vi "BUILD_install and upload core.vi"(6 "Buildlog":path, 8 "error in":errorcluster, 9 "args":string[](array[string]), 11 "vip built path":path) -> (0 "error out":errorcluster)   [LabVIEW 2010]
uses:
  <vilib>/JKI/VIPM API/VIPM API_vipm_api.lvlib
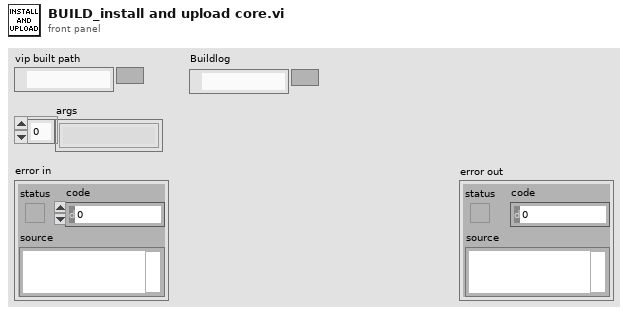
[diagram p1: front panel]
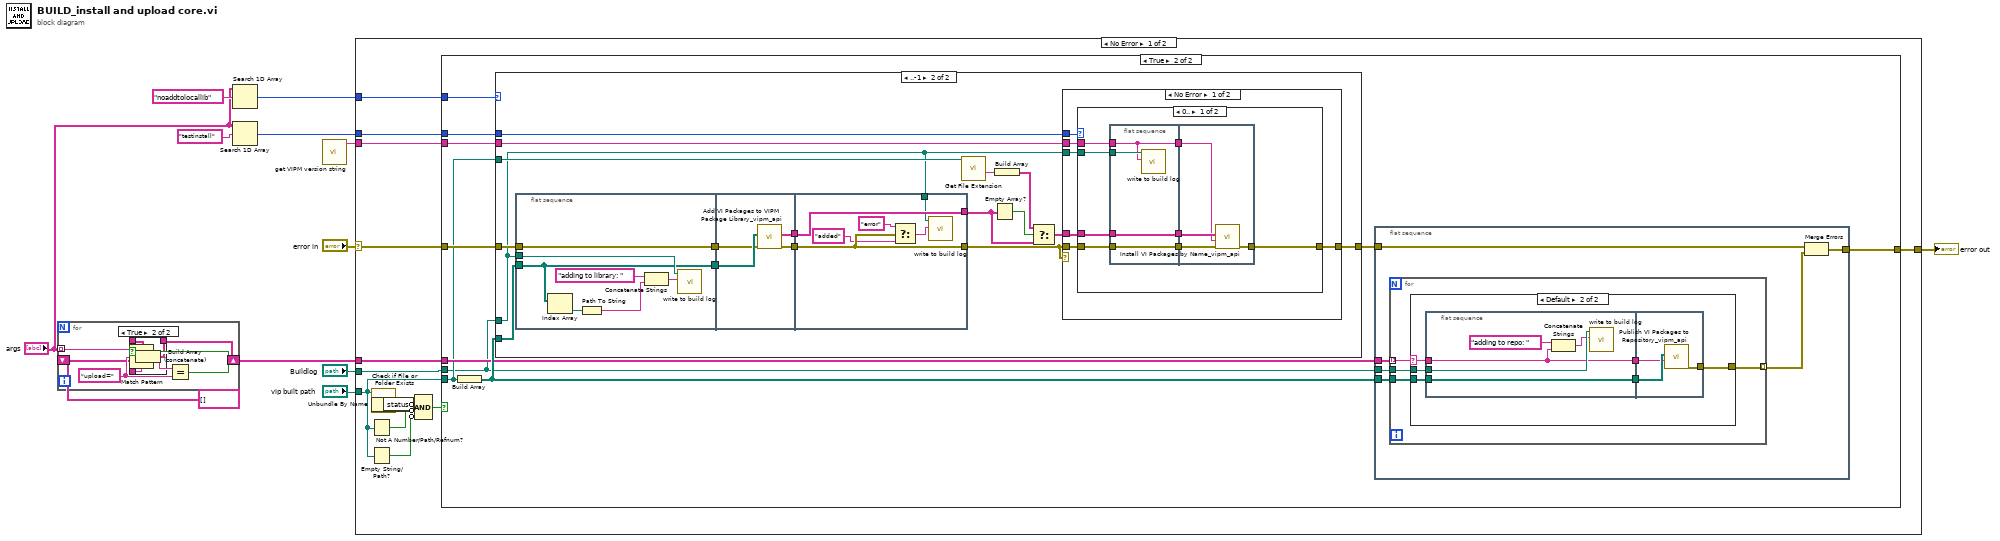
[diagram p0: block diagram]
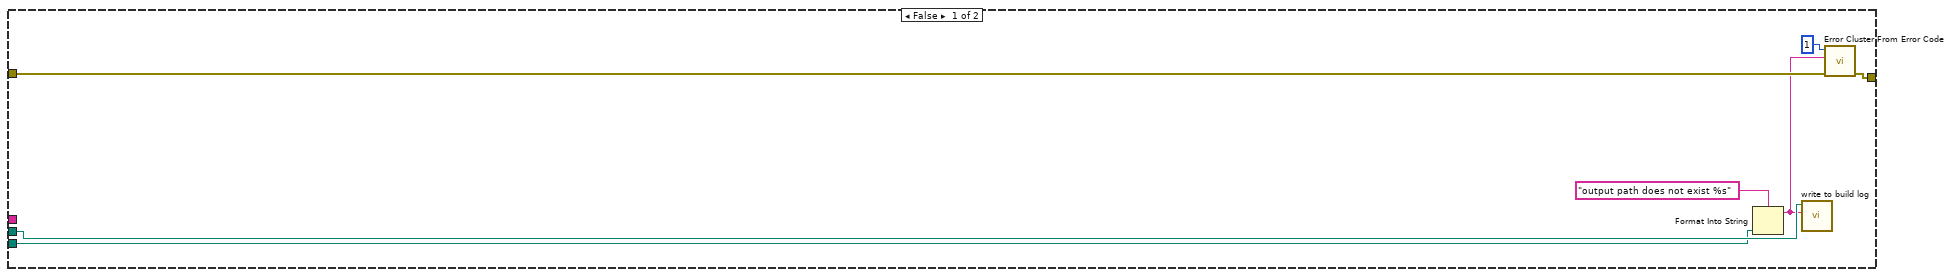
[diagram p3: hidden frame]
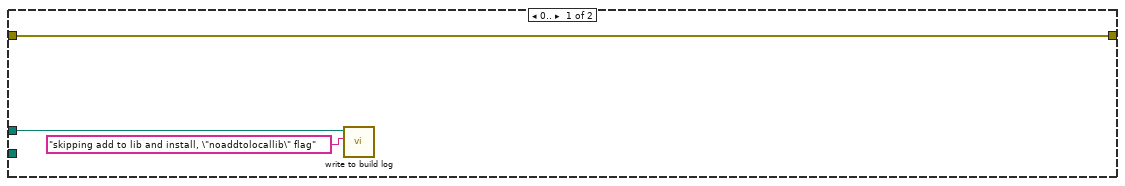
[diagram p4: hidden frame]
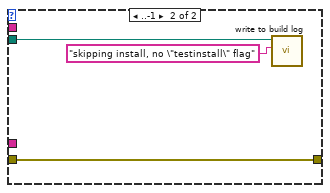
[diagram p5: hidden frame]
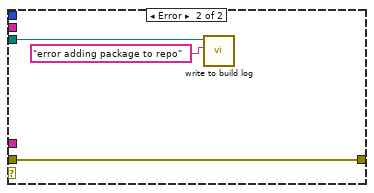
[diagram p6: hidden frame]
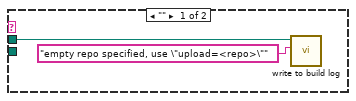
[diagram p7: hidden frame]
diagram:
  n1 = for {
    tunnel: "args" -> [w19] mode=indexing
    shift-right: [w13] -> w5
    shift-left: string[] [] ("Array") -> [w14]
    w17 = "upload=" ("regular expression")
    n2 = Match Pattern(string=w19, regular expression=w17) -> (match substring=w18:string, after substring=w16:string)  [unwired: 1 in, 2 out]
    n3 = Equal?(x=w18, y=w17) -> (x = y?=w15:bool)
    n4 = case shown="True" w15 {
      tunnel: w14 -> [w20 w22]
      tunnel: w16 -> [_ w21]
      tunnel: [w20 w23] -> w13
      frame False {
      }
      frame True {
        n5 = Build Array (concatenate)(w22, w21) -> (w23:string[])
      }
    }
  }
  n6 = Search 1D Array(1D array="args", element="noaddtolocallib") -> (index of element=w2:i32)  [unwired: 1 in]
  n7 = Search 1D Array(1D array="args", element="testinstall") -> (index of element=w6:i32)  [unwired: 1 in]
  n8 = call "get VIPM version string.vi"() -> ("version string"=w9:string)  [unwired: 11 in]
  n9 = case shown="No Error" "error in" {
    selector: "error in" -> [w35 w146]
    tunnel: "vip built path" -> [w27 _]
    tunnel: w9 -> [w37 _]
    tunnel: [w36 w146] -> w11
    tunnel: "Buildlog" -> [w34 _]
    tunnel: w6 -> [w33 _]
    tunnel: w5 -> [w32 _]
    tunnel: w2 -> [w25 _]
    frame No Error {
      n10 = Not A Number/Path/Refnum?(number/path/refnum=w27) -> (NaN/Path/Refnum?=w29:bool)
      n11 = Empty String/Path?(string/path=w27) -> (empty?=w28:bool)
      n12 = call <vilib>:"Check if File or Folder Exists.vi"("path"=w27) -> ("error out"=w30:errorcluster, "file or folder exists?"=w31:bool)  [unwired: 8 in, 1 out]
      n13 = Unbundle By Name(w30) -> ("status"=w24:bool)
      n14 = Compound Arithmetic op=AND(w31, invert w24, invert w29, invert w28) -> (w26:bool)
      n15 = case shown="True" w26 {
        tunnel: w27 -> [w42 w47]
        tunnel: [w40 w53] -> w36
        tunnel: w37 -> [_ w52]
        tunnel: w35 -> [w44 w50]
        tunnel: w34 -> [w43 w46]
        tunnel: w33 -> [_ w49]
        tunnel: w32 -> [_ w48]
        tunnel: w25 -> [_ w45]
        frame False {
          n16 = Format Into String(format string="output path does not exist %s", w42) -> (resulting string=w38:string)  [unwired: 2 in, 1 out]
          n17 = call "write to build log.vi"("text"=w38, "log"=w43) -> ()  [unwired: 10 in]
          n18 = call <vilib>:"Error Cluster From Error Code.vi"("error in (no error)"=w44, "error message (\"\")"=w38, "error code (0)"=1) -> ("error out"=w40:errorcluster)  [unwired: 6 in]
        }
        frame True {
          n19 = Build Array(w47) -> (w54:path[])
          n20 = case shown="..-1" w45 {
            tunnel: w54 -> [_ w70]
            tunnel: w52 -> [_ w69]
            tunnel: [w55 w68] -> w51
            tunnel: w50 -> [w55 w61]
            tunnel: w49 -> [_ w60]
            tunnel: w47 -> [_ w59]
            tunnel: w46 -> [w56 w58]
            frame 0.. {
              n21 = call "write to build log.vi"("text"="skipping add to lib and install, \"noaddtolocallib\" flag", "log"=w56) -> ()  [unwired: 10 in]
            }
            frame ..-1 {
              n22 = flat-sequence {
                tunnel: w61 -> [w81]
                tunnel: w70 -> [w75]
                tunnel: [w75] -> w74
                tunnel: [w81] -> w73
                tunnel: w58 -> [w80]
                tunnel: [w84] -> w72
                tunnel: [w83] -> w71
                tunnel: w74 -> [w85]
                tunnel: w73 -> [w82]
                tunnel: [w91] -> w65
                tunnel: [w90] -> w67
                tunnel: w72 -> [w90]
                tunnel: w71 -> [w91]
                tunnel: w58 -> [w86]
                frame #0 {
                  n23 = Index Array(array=w75) -> (element=w76:path)  [unwired: 1 in]
                  n24 = Path To String(path=w76) -> (string=w77:string)
                  n25 = Concatenate Strings("adding to library: " ("string"), w77) -> (w78:string)
                  n26 = call "write to build log.vi"("text"=w78, "log"=w80) -> ()  [unwired: 10 in]
                }
                frame #1 {
                  n27 = call <vilib>:"Add VI Packages to VIPM Package Library_vipm_api.vi"("error in (no error)"=w82, "Packages to add to VIPM Library (vipc,vip,ogp)"=w85) -> ("error out"=w84:errorcluster, "Package Names Added"=w83:string[])  [unwired: 8 in]
                }
                frame #2 {
                  n28 = Select(t="error" ("string"), s=w90, f="added" ("string")) -> (s? t:f=w87:string)
                  n29 = call "write to build log.vi"("text"=w87, "log"=w86) -> ()  [unwired: 10 in]
                }
              }
              n30 = call <vilib>:"Get File Extension.vi"("file"=w59) -> ("filename without extension"=w63:string)  [unwired: 7 in, 3 out]
              n31 = Empty Array?(array=w65) -> (empty?=w66:bool)
              n32 = Build Array(w63) -> (w62:string[])
              n33 = Select(t=w62, s=w66, f=w65) -> (s? t:f=w64:string[])
              n34 = case shown="No Error" w67 {
                tunnel: w67 -> [w97 w119]
                tunnel: w64 -> [w96 _]
                tunnel: w69 -> [w95 _]
                tunnel: [w94 w119] -> w68
                tunnel: w58 -> [w92 w118]
                tunnel: w60 -> [w93 _]
                frame No Error {
                  n35 = case shown="0.." w93 {
                    tunnel: w97 -> [w105 w116]
                    tunnel: w96 -> [w104 _]
                    tunnel: w95 -> [w103 _]
                    tunnel: [w102 w116] -> w94
                    tunnel: w92 -> [w98 w115]
                    frame 0.. {
                      n36 = flat-sequence {
                        tunnel: w103 -> [w106]
                        tunnel: w104 -> [w108]
                        tunnel: w105 -> [w109]
                        tunnel: [w109] -> w101
                        tunnel: [w108] -> w100
                        tunnel: [w106] -> w99
                        tunnel: w98 -> [w107]
                        tunnel: [w110] -> w102
                        tunnel: w101 -> [w113]
                        tunnel: w100 -> [w112]
                        tunnel: w99 -> [w111]
                        frame #0 {
                          n37 = call "write to build log.vi"("text"=w106, "log"=w107) -> ()  [unwired: 10 in]
                        }
                        frame #1 {
                          n38 = call <vilib>:"Install VI Packages by Name_vipm_api.vi"("error in (no error)"=w113, "LabVIEW Version"=w111, "Package Names to Install []"=w112) -> ("error out"=w110:errorcluster)  [unwired: 8 in]
                        }
                      }
                    }
                    frame ..-1 {
                      n39 = call "write to build log.vi"("text"="skipping install, no \"testinstall\" flag", "log"=w115) -> ()  [unwired: 10 in]
                    }
                  }
                }
                frame Error {
                  n40 = call "write to build log.vi"("text"="error adding package to repo", "log"=w118) -> ()  [unwired: 10 in]
                }
              }
            }
          }
          n41 = flat-sequence {
            tunnel: w54 -> [w125]
            tunnel: [w124] -> w53
            tunnel: w51 -> [w120]
            tunnel: w48 -> [w123]
            tunnel: w46 -> [w122]
            frame #0 {
              n42 = for {
                tunnel: w125 -> [w129]
                tunnel: [w128] -> w121 mode=indexing
                tunnel: w123 -> [w127] mode=indexing
                tunnel: w122 -> [w126]
                n43 = case shown="Default" w127 {
                  selector: w127 -> [_ w135]
                  tunnel: w129 -> [_ w137]
                  tunnel: [_ w136] -> w128
                  tunnel: w126 -> [w131 w132]
                  frame "" {
                    n44 = call "write to build log.vi"("text"="empty repo specified, use \"upload=<repo>\"", "log"=w131) -> ()  [unwired: 10 in]
                  }
                  frame Default {
                    n45 = flat-sequence {
                      tunnel: w135 -> [w139]
                      tunnel: w137 -> [w142]
                      tunnel: [w142] -> w134
                      tunnel: [w139] -> w133
                      tunnel: w132 -> [w141]
                      tunnel: [w144] -> w136
                      tunnel: w134 -> [w145]
                      tunnel: w133 -> [w143]
                      frame #0 {
                        n46 = Concatenate Strings("adding to repo: " ("string"), w139) -> (w140:string)
                        n47 = call "write to build log.vi"("text"=w140, "log"=w141) -> ()  [unwired: 10 in]
                      }
                      frame #1 {
                        n48 = call <vilib>:"Publish VI Packages to Repository_vipm_api.vi"("Repository Name"=w143, "Packages to publish to Repository Library (vip,ogp)"=w145) -> ("error out"=w144:errorcluster)  [unwired: 8 in, 1 out]
                      }
                    }
                  }
                }
              }
              n49 = Merge Errors(w120, w121) -> (w124:errorcluster)
            }
          }
        }
      }
    }
    frame Error {
    }
  }
  "error out" <- w11
